vi "Cmd_Edges.vi"(4 "Rising Only":bool, 8 "Devices":string[](array[string]), 9 "Prev":bool[](array[boolean]), 10 "Bits":bool[](array[boolean]), 11 "Queue":refnum<queue>) -> ()   [LabVIEW 2026]
doc: "Use this template to build a VI to use as a subVI."
panel:
  # "ÕfÃ÷£º°´âoêÁÐºÍÉÏÒ»È¦±ÈÝ^£¬ÓÐ×»¯²Å·ÅßMÐÁÐ¡£Rising Only\n é True rÖ»ËÍ°´ÏÂ£¬·Åé_²»ËÍ¡£"
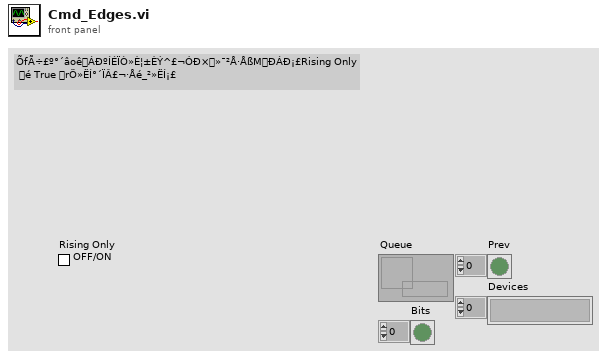
[diagram p1: front panel]
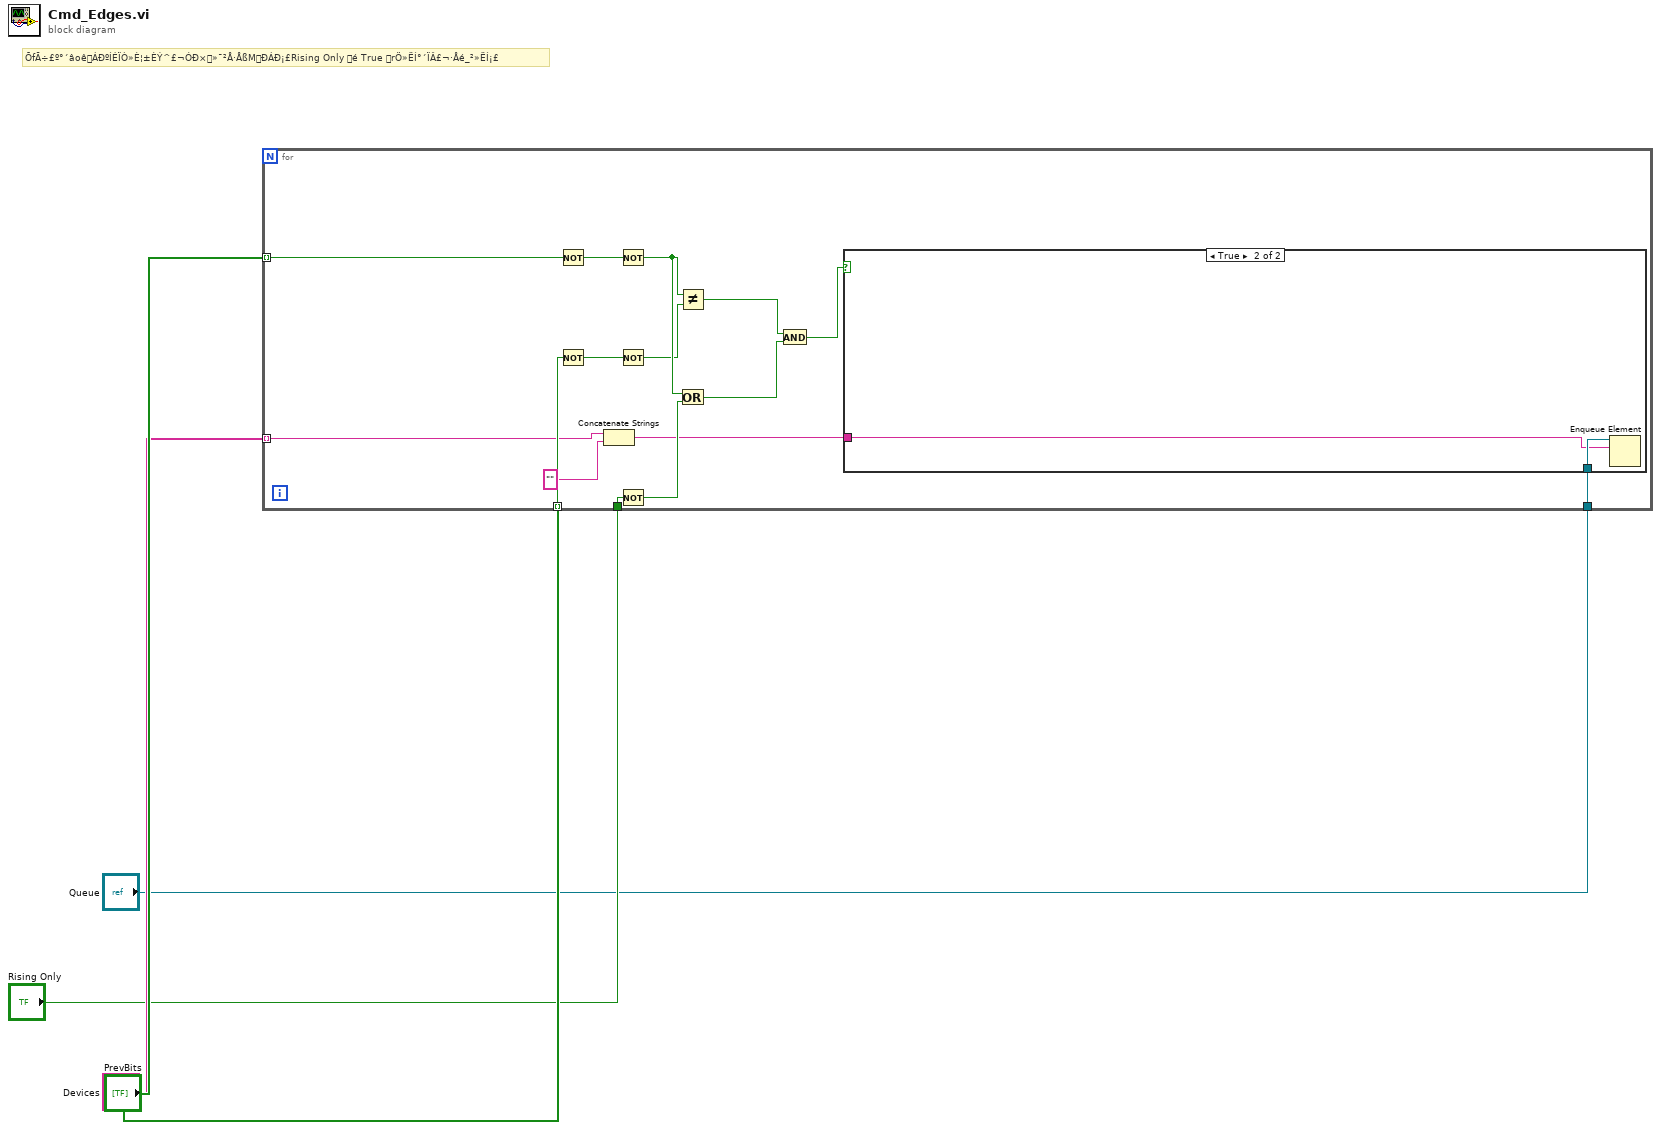
[diagram p0: block diagram]
diagram:
  # "ÕfÃ÷£º°´âoêÁÐºÍÉÏÒ»È¦±ÈÝ^£¬ÓÐ×»¯²Å·ÅßMÐÁÐ¡£Rising Only é True rÖ»ËÍ°´ÏÂ£¬·Åé_²»ËÍ¡£"
  n1 = for {
    tunnel: "Bits" -> [w20] mode=indexing
    tunnel: "Prev" -> [w18] mode=indexing
    tunnel: "Devices" -> [w16] mode=indexing
    tunnel: "Rising Only" -> [w12]
    tunnel: "Queue" -> [w7]
    n2 = Not(x=w20) -> (.not. x?=w19:bool)
    n3 = Not(x=w18) -> (.not. x?=w17:bool)
    n4 = Concatenate Strings(w16, "") -> (w6:string)
    n5 = Not(x=w19) -> (.not. x?=w14:bool)
    n6 = Not(x=w17) -> (.not. x?=w13:bool)
    n7 = Not(x=w12) -> (.not. x?=w11:bool)
    n8 = Not Equal?(x=w14, y=w13) -> (x != y?=w10:bool)
    n9 = Or(x=w14, y=w11) -> (x .or. y?=w9:bool)
    n10 = And(x=w10, y=w9) -> (x .and. y?=w8:bool)
    n11 = case shown="True" w8 {
      tunnel: w7 -> [_ w22]
      tunnel: w6 -> [_ w21]
      frame False {
      }
      frame True {
        n12 = Enqueue Element(queue=w22, element=w21) -> ()  [unwired: 2 in, 3 out]
      }
    }
  }
